vi "Run Measurement.vi"(8 "error in (no error)":errorcluster, 11 "Operator UI in":refnum<class "Measurement UI.lvclass">) -> (0 "error out":errorcluster, 3 "Operator UI out":refnum<class "Measurement UI.lvclass">)   [LabVIEW 2017, in "Measurement UI.lvlib" / "Measurement UI.lvclass"]
uses:
  Measurement UI.lvclass
  C:/Program Files (x86)/National Instruments/LabVIEW 2017/vi.lib/ActorFramework/Actor/Actor.lvclass
  <vilib>/ActorFramework/Actor/Actor.lvclass/Actor.ctl
  <vilib>/ActorFramework/Message Enqueuer/Message Enqueuer.lvclass/Message Enqueuer.ctl
  <vilib>/ActorFramework/Message Enqueuer/Init from Existing Queue.vi
  <vilib>/ActorFramework/Message Enqueuer/Message Enqueuer.lvclass
  Controller/Messages/Launch Measurements Message/Launch Measurements Message.lvclass
  User Interface/Messages/Update Status Display/Update Status Display.lvclass
  <vilib>/ActorFramework/Actor/Actor.lvclass
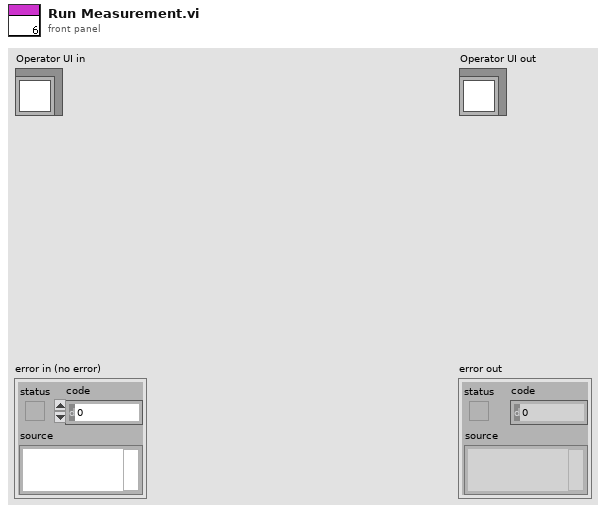
[diagram p1: front panel]
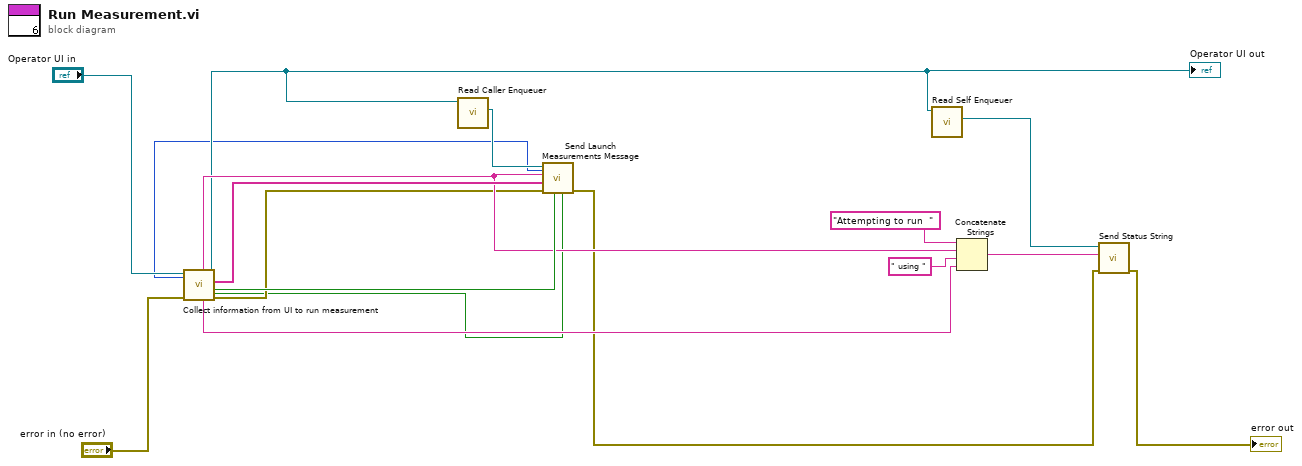
[diagram p0: block diagram]
diagram:
  n1 = call "Collect information from UI to run measurement.vi"("error in (no error)"="error in (no error)", "Measurement UI in"="Operator UI in") -> ("error out"=w5:errorcluster, "Show UI?"=w16:bool, "Device Names"=w17:string[], "Measurement UI out"=w7:refnum<class "Measurement UI.lvclass">, "String"=w11:string, "Measurement Name"=w14:string, "Run continuously?"=w2:bool, "Iterations"=w1:i32)  [unwired: 2 in]
  "Operator UI out" <- w7
  n2 = call <vilib>:"Read Caller Enqueuer.vi"("Actor"=w7) -> ("Caller Enqueuer"=w10:refnum<class "Message Enqueuer.lvclass">)  [unwired: 10 in]
  n3 = call "Send Launch Measurements Message.vi"("Continuous Run"=w2, "Show FP?"=w16, "Iterations"=w1, "error in (no error)"=w5, "Device Names"=w17, "Measurement Name"=w14, "Self Enqueuer In"=w10) -> ("error out"=w4:errorcluster)  [unwired: 3 in, 1 out]
  n4 = call <vilib>:"Read Self Enqueuer.vi"("Actor"=w7) -> ("Self Enqueuer"=w9:refnum<class "Message Enqueuer.lvclass">)  [unwired: 10 in]
  n5 = Concatenate Strings("Attempting to run  " ("string"), w14, " using " ("string"), w11) -> (w12:string)
  n6 = call "Send Status String.vi"("error in (no error)"=w4, "String"=w12, "Message Enqueuer in"=w9) -> ("error out"=→"error out":errorcluster)  [unwired: 7 in, 1 out]
